vi "NR Change RB Status.vi"(8 "error in (no error)":errorcluster caption="에러 입력(에러 없음)", 9 "RB Offset":i32, 10 "RB Size":i32, 11 "Instrument Manager 입력":refnum<class "Instrument Manager.lvclass">) -> (0 "error out":errorcluster caption="에러 출력", 3 "Instrument Manager 출력":refnum<class "Instrument Manager.lvclass">)   [LabVIEW 2023, in "Instrument Manager.lvclass"]
uses:
  Instrument Manager.lvclass
  Instrument Manager.lvclass/Instrument Manager.ctl
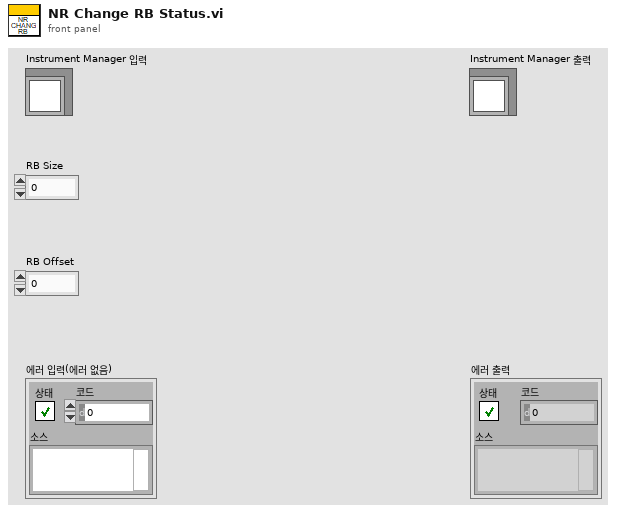
[diagram p1: front panel]
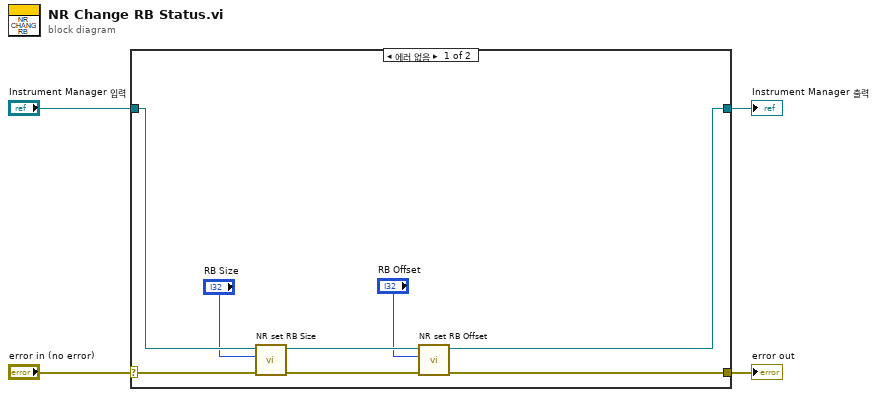
[diagram p0: block diagram]
diagram:
  n1 = case shown="에러 없음" "error in (no error)" {
    selector: "error in (no error)" -> [w12 w14]
    tunnel: [w10 w14] -> w3
    tunnel: [w7 w13] -> w1
    tunnel: "Instrument Manager 입력" -> [w9 w13]
    frame No Error {
      n2 = call "NR set RB Size.vi"("error in (no error)"=w12, "RB Value (0~273)"="RB Size", "Instrument Manager 입력"=w9) -> ("error out"=w11:errorcluster, "Instrument Manager 출력"=w8:refnum<class "Instrument Manager.lvclass">)  [unwired: 7 in]
      n3 = call "NR set RB Offset.vi"("error in (no error)"=w11, "RB Value (0~273)"="RB Offset", "Instrument Manager 입력"=w8) -> ("error out"=w10:errorcluster, "Instrument Manager 출력"=w7:refnum<class "Instrument Manager.lvclass">)  [unwired: 7 in]
    }
    frame Error {
    }
  }
  "error out" <- w3
  "Instrument Manager 출력" <- w1
